vi "Create Message Data Cluster.vi"(6 "generate serialization helpers":bool, 7 "owning typedef":refnum<vi>, 8 "error in (no error)":errorcluster, 9 "library in":refnum<vi>, 10 "message element metafata":T1[](array[typedef]), 11 "cluster in":refnum<vi>) -> (0 "error out":errorcluster, 1 "library out":refnum<vi>, 3 "cluster out":refnum<vi>)   [LabVIEW 2019, in "gRPC Template Creation Utility.lvlib"]
uses:
  gRPC Template Creation Utility.lvlib
  TypeDefs/Message Element Metadata (Scripting).ctl
  TypeDefs/Message Element Type.ctl
  <vilib>/Utility/miscctls.llb/LVPositionTypeDef.ctl
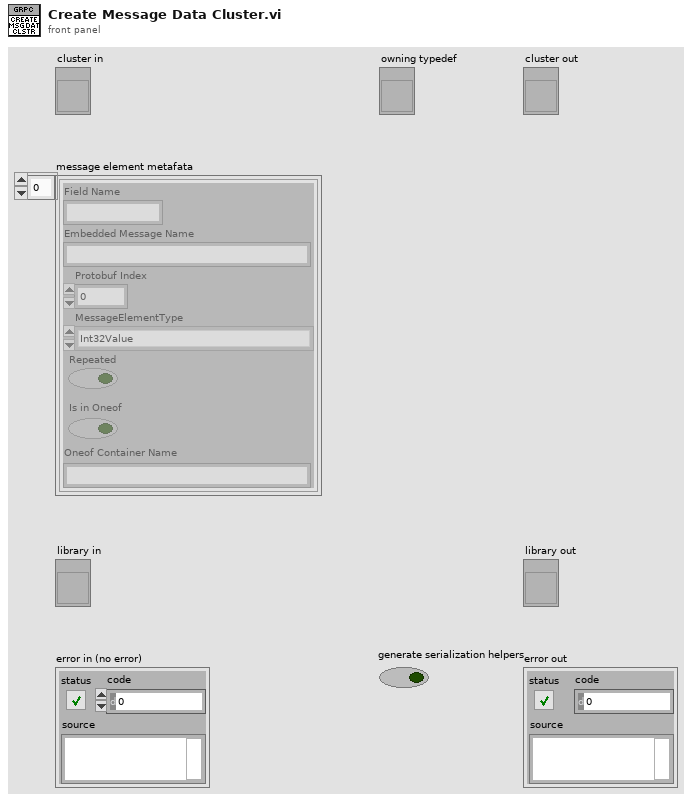
[diagram p1: front panel]
types:
  T1 = typedef "gRPC Template Creation Utility.lvlib/Message Element Metadata (Scripting).ctl" = cluster{"Field Name":string, "Embedded Message Name":string, "Protobuf Index":i32, "MessageElementType":T2, "Repeated":bool, "Is in Oneof":bool, "Oneof Container Name":string}
  T2 = typedef "gRPC Template Creation Utility.lvlib/Message Element Type.ctl" = enum32{"Int32Value", "FloatValue", "DoubleValue", "BoolValue", "StringValue", "MessageValue", "Int64Value", "UInt32Value", "UInt64Value", "EnumValue", "Bytes", "Fixed64", "Fixed32", "SFixed64", "SFixed32", "SInt64", "SInt32"}
  T3 = typedef "LVPositionTypeDef.ctl" = cluster{"Left":i32, "Top":i32}
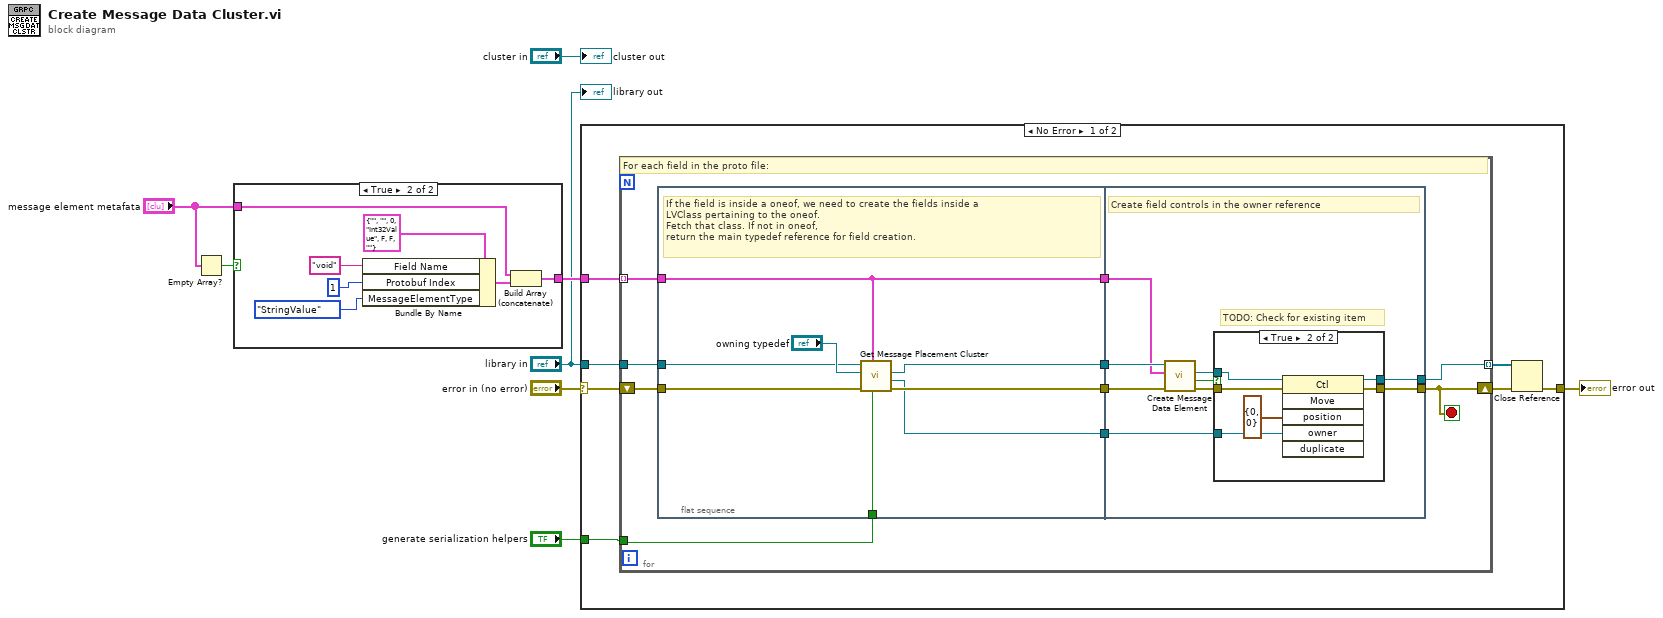
[diagram p0: block diagram]
diagram:
  n1 = Empty Array?(array="message element metafata") -> (empty?=w5:bool)
  n2 = case shown="True" w5 {
    tunnel: "message element metafata" -> [w9 w16]
    tunnel: [w9 w15] -> w4
    frame False {
    }
    frame True {
      n3 = Bundle By Name(cluster=T1 {"Field Name"="", "Embedded Message Name"="", "Protobuf Index"=0, "MessageElementType"=enum."Int32Value", "Repeated"=FALSE, "Is in Oneof"=FALSE, "Oneof Container Name"=""} ("MessageElementMetadata"), "Field Name"="void", "Protobuf Index"=1, "MessageElementType"=Message_Element_Type."StringValue") -> (w10:T1)
      n4 = Build Array (concatenate)(w16, w10) -> (w15:T1[])
    }
  }
  n5 = case shown="No Error" "error in (no error)" {
    selector: "error in (no error)" -> [w19 w59]
    tunnel: [w17 w59] -> w8
    tunnel: "library in" -> [w21 _]
    tunnel: w4 -> [w20 _]
    tunnel: "generate serialization helpers" -> [w18 _]
    frame No Error {
      n6 = for {
        tunnel: [w29] -> w23 mode=indexing
        shift-right: [w24] -> w22
        shift-left: w19 -> [w33]
        tunnel: w20 -> [w30] mode=indexing
        tunnel: w21 -> [w32]
        tunnel: w18 -> [w28]
        stop <- w24 stop-if-true
        # "For each field in the proto file:"
        n7 = flat-sequence {
          tunnel: w30 -> [w34]
          tunnel: w33 -> [w41]
          tunnel: w32 -> [w37]
          tunnel: [w40] -> w31
          tunnel: w28 -> [w39]
          tunnel: [w36] -> w27
          tunnel: [w35] -> w26
          tunnel: [w34] -> w25
          tunnel: w31 -> [w50]
          tunnel: w27 -> [w49]
          tunnel: w26 -> [w44]
          tunnel: w25 -> [w43]
          tunnel: [w48] -> w29
          tunnel: [w42] -> w24
          frame #0 {
            # "If the field is inside a oneof, we need to create the fields inside a \nLVClass pertaining to the oneof. \nFetch that class. If not in oneof, \nreturn the main typedef reference for field creation."
            n8 = call "Get Message Placement Cluster.vi"("Is Serialization Cluster"=w39, "MessageElementMetadata"=w34, "error in (no error)"=w41, "VI in"="owning typedef", "Library"=w37) -> ("error out"=w40:errorcluster, "Control ref out"=w36:refnum<vi>, "VI out"=w35:refnum<vi>)  [unwired: 2 in, 2 out]
          }
          frame #1 {
            # "TODO: Check for existing item"
            # "Create field controls in the owner reference"
            n9 = call "Create Message Data Element.vi"("error in (no error)"=w50, "message element metadata"=w43, "owning vi in"=w44) -> ("error out"=w45:errorcluster, "data element created"=w47:bool, "data element control"=w46:refnum<vi>)  [unwired: 4 in, 2 out]
            n10 = case shown="True" w47 {
              tunnel: w49 -> [_ w58]
              tunnel: [w52 w57] -> w48
              tunnel: w46 -> [w52 w55]
              tunnel: w45 -> [w51 w54]
              tunnel: [w51 w53] -> w42
              frame False {
              }
              frame True {
                n11 = invoke class="Ctl" method="Move"(reference=w55, error in=w54, "position"=T3 {"Left"=0, "Top"=0}, "owner"=w58) -> (reference out=w57:refnum<vi>, error out=w53:errorcluster)  [unwired: 2 in, 4 out]
              }
            }
          }
        }
      }
      n12 = Close Reference(reference=w23, error in (no error)=w22) -> (error out=w17:errorcluster)
    }
    frame Error {
    }
  }
  "error out" <- w8
  "cluster out" <- "cluster in"
  "library out" <- "library in"
